vi "VIH HelpGen - HREF - Build.vi"(8 "Text to enclose":string, 10 "Tree Item Tag":string, 11 "File Path":path) -> (3 "A HREF":string)   [LabVIEW 2014]
doc: "::: VI Helpeks :::\nCopyright (c) 2000-2026 Konstantin Shifershteyn. All rights reserved."
panel:
  # "VI Helpeks\nCopyright (c) 2012-2026 Konstantin Shifershteyn"
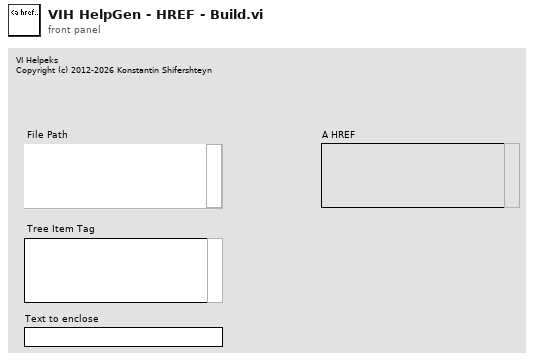
[diagram p1: front panel]
types:
  T1 = typedef "VIH Project Tree Typedef - Tree Item Type.ctl" = enum32{"<Invalid>", "Project", "Proj Files", "Proj Rules", "File Group", "Rule Group", "Any File", "LV Func", ".mnu", ".mnu (dyn)", ".vi", ".vi (dyn)", ".vit", ".vit (dyn)", ".ctl", ".ctl (dyn)", ".ctt", ".ctt (dyn)", "polyVI", "polyVI (dyn)", "expVI", "expVI (dyn)", "HTML", "PolyVI Inst"}
  T2 = typedef "VIH HelpGen Typedef - Palette - Item Type Enum.ctl" = enum32{"<Invalid>", "<unknown>", "VI", "Menu", "LV Func", "Express VI", "Poly VI", "CTL", "HTML"}
  T3 = typedef "Palette Menu.lvlib/Palette Data.ctl" = cluster{"display name":string, "view format":T4, "palette width":i16, "items":T5, "256 color icon":picture, "B&W color icon":picture, "help information":T7, "palette description":string, "synchronize information":T8}
  T4 = typedef "Palette Menu.lvlib/View Format.ctl" = u16
  T5 = typedef "Palette Menu.lvlib/Items.ctl" = T6[]
  T6 = typedef "Palette Menu.lvlib/Item.ctl" = cluster{"item path":path, "library path (.lvlib)":path, "use default lvlib palette":bool, "short name":string, "place VI contents":bool, "hide synchronized item":bool, "reserve spot for synch item":bool, "configure when placing VI contents":bool}
  T7 = typedef "Palette Menu.lvlib/Help Info.ctl" = cluster{"help tag":string, "help file path ":path}
  T8 = typedef "Palette Menu.lvlib/Synchronize Info.ctl" = cluster{"synchronize with directory":bool, "synchronize directory path":path}
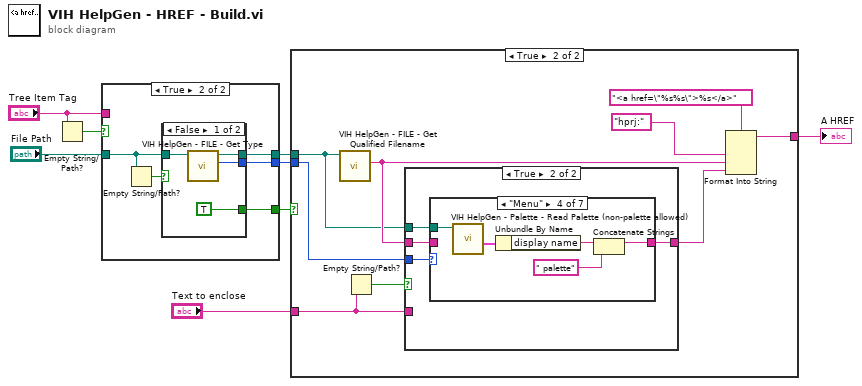
[diagram p0: block diagram]
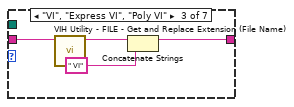
[diagram p6: hidden frame]
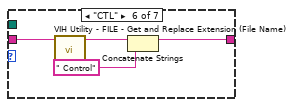
[diagram p8: hidden frame]
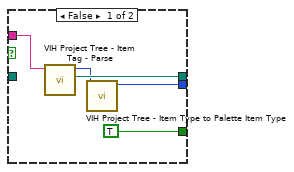
[diagram p10: hidden frame]
diagram:
  n1 = Empty String/Path?(string/path="Tree Item Tag") -> (empty?=w7:bool)
  n2 = case shown="True" w7 {
    tunnel: [w13 w18] -> w4
    tunnel: "Tree Item Tag" -> [w12 _]
    tunnel: "File Path" -> [_ w15]
    tunnel: [w11 w17] -> w5
    tunnel: [TRUE w14] -> w2
    frame False {
      n3 = call "VIH Project Tree - Item Tag - Parse.vi"("Tree Item Tag"=w12) -> ("Item File Path"=w13:path, "Item Type"=w10:T1)  [unwired: 8 in, 1 out]
      n4 = call "VIH Project Tree - Item Type to Palette Item Type.vi"("Tree Item Type"=w10) -> ("Item/File Type"=w11:T2)  [unwired: 9 in, 1 out]
    }
    frame True {
      n5 = Empty String/Path?(string/path=w15) -> (empty?=w16:bool)
      n6 = case shown="False" w16 {
        tunnel: w15 -> [w22 w23]
        tunnel: [w21 w23] -> w18
        tunnel: [w20 _] -> w17
        tunnel: [TRUE _] -> w14
        frame False {
          n7 = call "VIH HelpGen - FILE - Get Type.vi"("File Path"=w22) -> ("File Type"=w20:T2, "dup File Path"=w21:path)  [unwired: 8 in, 1 out]
        }
        frame True {
        }
      }
    }
  }
  n8 = case shown="True" w2 {
    tunnel: w5 -> [_ w30]
    tunnel: w4 -> [_ w24]
    tunnel: [_ w29] -> w3
    tunnel: "Text to enclose" -> [_ w26]
    frame False {
    }
    frame True {
      n9 = call "VIH HelpGen - FILE - Get Qualified Filename.vi"("File Path"=w24) -> ("Qualified name"=w25:string)  [unwired: 9 in, 1 out]
      n10 = Empty String/Path?(string/path=w26) -> (empty?=w28:bool)
      n11 = case shown="True" w28 {
        tunnel: w30 -> [_ w37]
        tunnel: w25 -> [_ w36]
        tunnel: w24 -> [_ w35]
        tunnel: [w33 w34] -> w27
        tunnel: w26 -> [w33 _]
        frame False {
        }
        frame True {
          n12 = case shown="\"Menu\"" w37 {
            tunnel: w36 -> [w38 w39 w43 _ w49 w53 w54]
            tunnel: [w38 w39 w41 w47 w49 w51 w54] -> w34
            tunnel: w35 -> [_ _ _ w45 _ _ _]
            frame "<Invalid>" {
            }
            frame "<unknown>" {
            }
            frame "VI", "Express VI", "Poly VI" {
              n13 = call "VIH Utility - FILE - Get and Replace Extension (File Name).vi"("File name"=w43) -> ("File name out"=w42:string)  [unwired: 9 in, 1 out]
              n14 = Concatenate Strings(w42, " VI" ("string")) -> (w41:string)
            }
            frame "Menu" {
              n15 = call "VIH HelpGen - Palette - Read Palette (non-palette allowed).vi"("Palette Path"=w45) -> ("palette data"=w44:T3)  [unwired: 8 in, 2 out]
              n16 = Unbundle By Name(w44) -> ("display name"=w48:string)
              n17 = Concatenate Strings(w48, " palette" ("string")) -> (w47:string)
            }
            frame "LV Func" {
            }
            frame "CTL" {
              n18 = call "VIH Utility - FILE - Get and Replace Extension (File Name).vi"("File name"=w53) -> ("File name out"=w52:string)  [unwired: 9 in, 1 out]
              n19 = Concatenate Strings(w52, " Control" ("string")) -> (w51:string)
            }
            frame "HTML" {
            }
          }
        }
      }
      n20 = Format Into String(format string="<a href=\"%s%s\">%s</a>", "hprj:" ("input 1"), w25, w27) -> (resulting string=w29:string)  [unwired: 2 in, 1 out]
    }
  }
  "A HREF" <- w3
